vi "AR.Drone MAIN.vi"() -> ()   [LabVIEW 2014]
uses:
  Resources/Others/Control cluster.ctl
  <vilib>/LVH/AR Drone Toolkit/Decode NavData/Typedefs/NavData Demo.ctl
  Resources/Global.vi
  Kinect Extention/Kinect Global.vi
  <vilib>/LVH/AR Drone Toolkit/AR Drone.lvlib
panel:
  in  "Tab Control 3":enum32{"Flight Control"}(tab)
  in  "Manual":bool=TRUE
  in  "Switch control":bool
  in  "Enable Kinect Extention":bool
  in  "Tab Control 2":enum32{"Setup", "Debug&Test Info", "NavData"}(tab)
  in  "Enable Video":bool
  in  "Enable Controller Setup":bool
  in  "Reset OCR":bool
  in  "Secondary VI":u16(ring)=1 items=["Auto Hovering with Position Prediction.vi", "Simple Video.vi", "Circle detection.vi", "OCR Control.vi"]
  in  "Setup Parameters":T1={"Drone IP address"="192.168.1.1", "Home IP address"="192.168.1.2", "Flight Mode"=enum."INDOOR MODE", "Mounted Hull"=enum."INDOOR HULL", "Video Camera"=0, "Max Altitude (m)"=3.0, "Max Pitch and Roll Angle (deg)"=8.0, "Max Vertical Speed (m/s)"=0.7, "Max Yaw Speed (deg/s)"=100.0} {"Video Camera" items=["Bottom Camera"=1, "Front Camera"=0, "Front in Bottom"=3, "Bottom in Front"=2]}
  in  "Adjustments (affects Secondary VIs)":cluster{"Sensitivity":dbl, "Null Zone":dbl}={"Sensitivity"=1.0, "Null Zone"=1.0} {"Null Zone" scale=0.0..2.0; "Sensitivity" scale=0.0..2.0}
  in  "Enable Kinect Setup":bool
  out "Succesful Controller Setup":bool
  out "Succesful Drone Setup":bool
  in  "Control loop wait (ms)":u32=25
  out "Control loop Refesh Rate (ms)":u32
  in  "Video acquisition wait (ms)":u32=30
  out "Loop error":errorcluster
  out "Setup error":errorcluster
  out "Loop error (Ctr & Nav)":bool
  in  "Clear errors":bool
  out "Video procesing Refresh Rate (ms)":i32
  out "NavData Out":T2={"control state"=enum."INIT", "battery percentage"=100, "pitch (deg)"=0.0, "roll (deg)"=0.0, "yaw (deg)"=0.0, "altitude (cm)"=0, "vx (cm/s)?"=0.0, "vy (cm/s)?"=0.0, "vz (cm/s)?"=0.0, "detection cam type"=3}
  out "Battery Remaining":dbl(slide)=100.0 scale=0.0..100.0
  out "Hover (H)":bool
  out "Control Cluster":T3 {"Yaw Speed" scale=-1.0..1.0; "Vertical Speed" scale=-1.0..1.0; "Pitch" scale=-1.0..1.0; "Roll" scale=-1.0..1.0}
  out "Take off/Land (T)":bool
  in  "Tab Control":T4(tab)
  out "Raw":picture
  in  "Take photo":bool
  out "Generated path":path
  out "Error creating image":errorcluster
  out "Grayscale":T5(plugin-control)
  out "B&W":T5(plugin-control)
  in  "Calibrate Pitch":bool
  out "3D Picture":refnum<vi>(3d-picture)
  in  "stop":bool
  in  "Emergency Landing":bool
  # "Select Manual/Auto Control (based on Secondary VI)"
  # "Keyboard/Controller input"
  # "Enable Kinect gestuires (BETA)"
  # "(1 is default)"
  # "FOR ADVANCED USERS ONLY!"
  # "Not recommended!!!"
  # "This ignores the errors but does NOT eliminate them!"
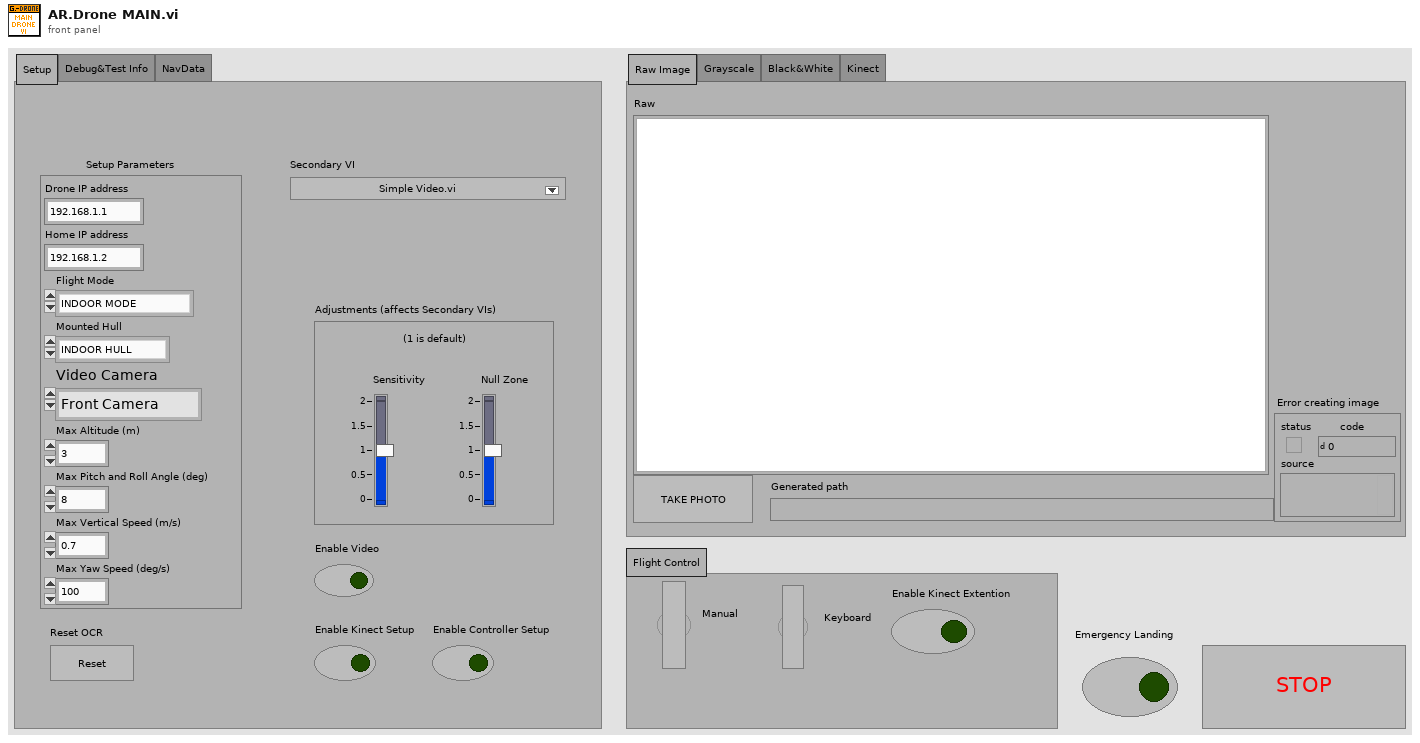
[diagram p1: front panel]
types:
  T1 = cluster{"Drone IP address":string, "Home IP address":string, "Flight Mode":enum8{"OUTDOOR MODE", "INDOOR MODE"}, "Mounted Hull":enum8{"OUTDOOR HULL", "INDOOR HULL"}, "Video Camera":u8, "Max Altitude (m)":sgl, "Max Pitch and Roll Angle (deg)":sgl, "Max Vertical Speed (m/s)":sgl, "Max Yaw Speed (deg/s)":sgl}
  T2 = typedef "AR Drone.lvlib/NavData Demo.ctl" = cluster{"control state":enum32{"DEFAULT", "INIT", "LANDING", "FLYING", "HOVERING", "TEST", "TRANS_TAKEOFF", "TRANS_GOTOFIX", "TRANS_LANDING"}, "battery percentage":u32, "pitch (deg)":sgl, "roll (deg)":sgl, "yaw (deg)":sgl, "altitude (cm)":u32, "vx (cm/s)?":sgl, "vy (cm/s)?":sgl, "vz (cm/s)?":sgl, "detection cam type":u32}
  T3 = typedef "Control cluster.ctl" = cluster{"Roll":sgl, "Pitch":sgl, "Vertical Speed":sgl, "Yaw Speed":sgl}
  T4 = enum32{"Raw Image", "Grayscale", "Black&White", "Kinect"}
  T5 = typedef "IMAQ Image.ctl" = refnum<image>
  T6 = typedef "imagedata.ctl" = cluster{"image type":i32, "image depth":i32, "image":u8[], "mask":u8[], "colors":u32[], "Rectangle":cluster{"left":i16, "top":i16, "right":i16, "bottom":i16}}
  T7 = typedef "AR Drone.lvlib/AR Drone Resource.ctl" = cluster{"UDP Control Connection":refnum<k16>, "UDP NavData Connection":refnum<k16>, "UDP Video Connection (Drone 1.0)":refnum<k16>, "TCP Video Connection (Drone 2.0)":refnum<k5>, "TCP Control Port Connection":refnum<k5>, "Drone IP address":string, "Drone Command Port":u16, "Drone NavData Port":u16, "Drone Vid Stream Port":u16, "Drone TCP Control Port":u16, "Home IP address":string, "Home Command Port":u16, "Home NavData Port":u16, "Home Vid Stream Port":u16, "Drone Version":i32, "Drone Index":i32, "Command Sequence":i32}
  T8 = cluster{"Roll":dbl, "Pitch":dbl, "Vertical Speed":dbl, "Yaw Speed":dbl}
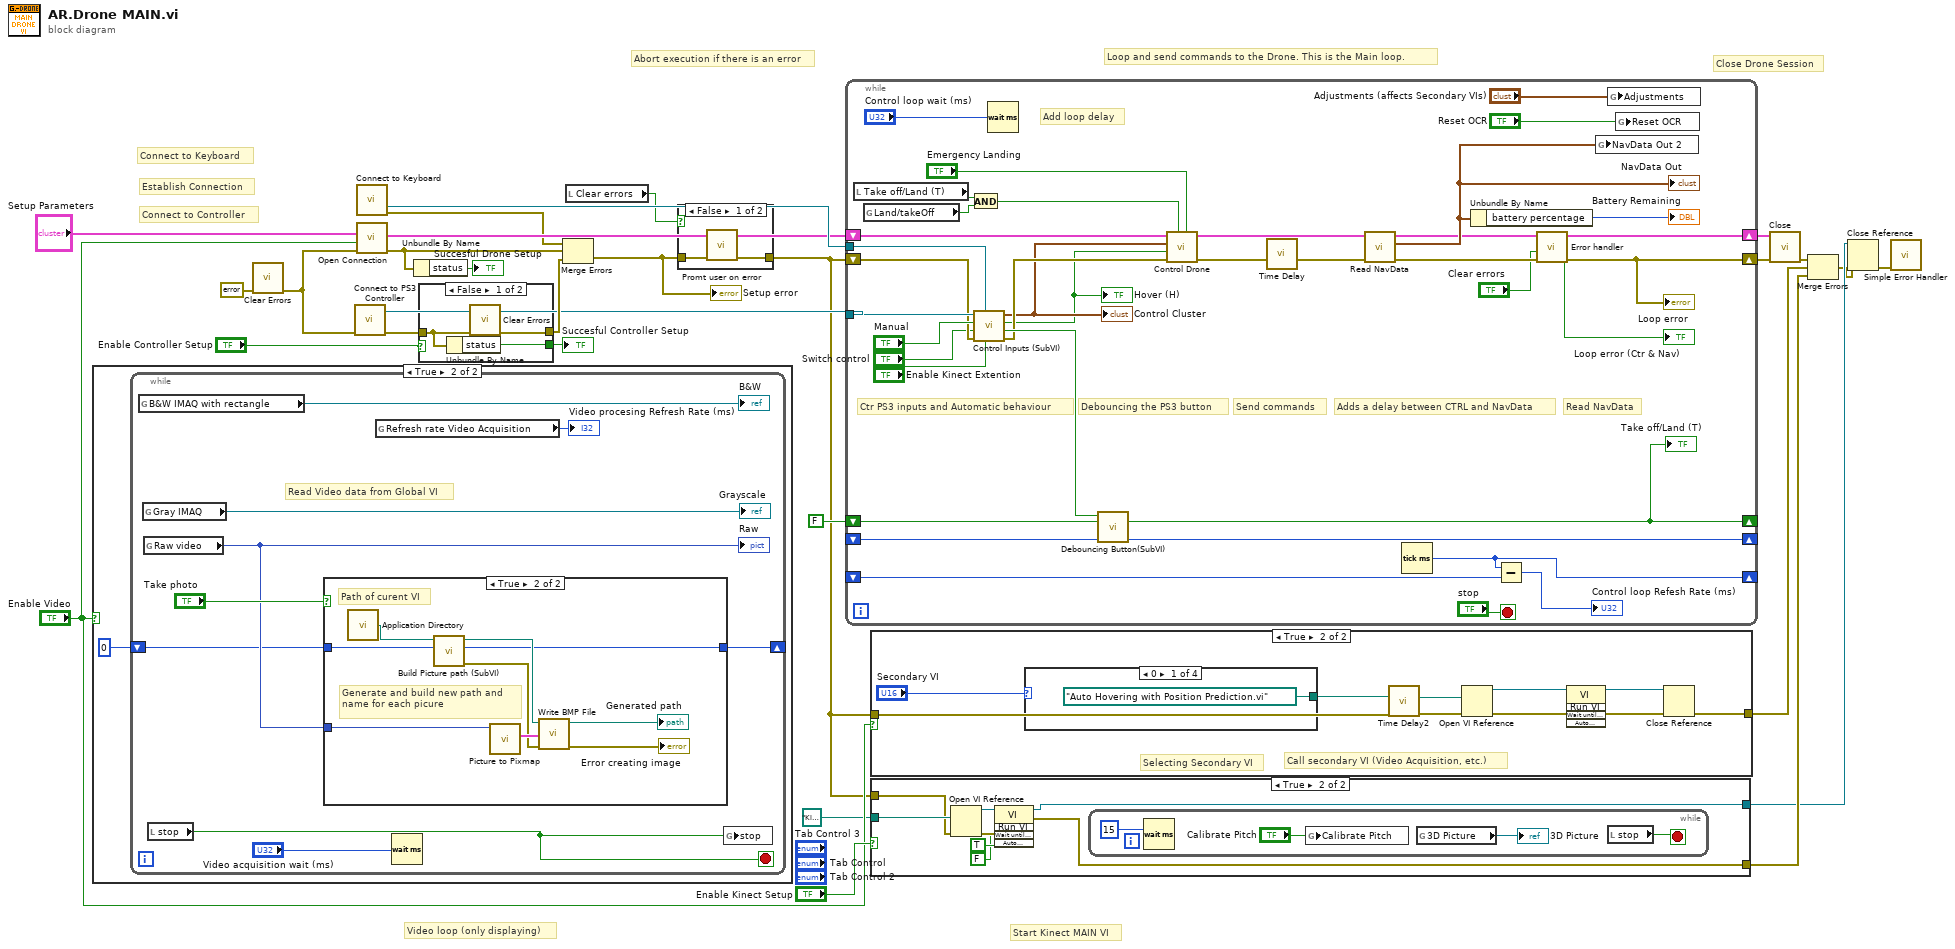
[diagram p0: block diagram]
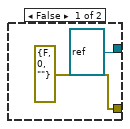
[diagram p2: hidden frame]
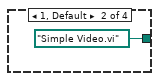
[diagram p4: hidden frame]
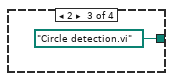
[diagram p5: hidden frame]
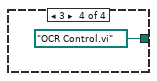
[diagram p6: hidden frame]
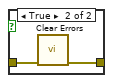
[diagram p9: hidden frame]
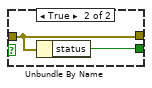
[diagram p10: hidden frame]
diagram:
  # "Start Kinect MAIN VI"
  # "Video loop (only displaying)"
  # "Connect to Keyboard"
  # "Connect to Controller"
  # "Abort execution if there is an error"
  # "Establish Connection"
  # "Close Drone Session"
  # "Loop and send commands to the Drone. This is the Main loop."
  n1 = case shown="True" "Enable Video" {
    frame False {
    }
    frame True {
      n2 = while {
        shift-right: [w31] -> _
        shift-left: 0 -> [w32]
        stop <- w38 stop-if-true
        # "Read Video data from Global VI"
        n3 = global read "Global.vi" "B&W IMAQ with rectangle"() -> (→"B&W":T5)
        n4 = global read "Global.vi" "Gray IMAQ"() -> (→"Grayscale":T5)
        n5 = global read "Global.vi" "Raw video"() -> (w33:picture)
        "Raw" <- w33
        n6 = local read "stop"() -> (w38:bool)
        n7 = case shown="True" "Take photo" {
          tunnel: w33 -> [_ w46]
          tunnel: w32 -> [w39 w44]
          tunnel: [w39 w43] -> w31
          frame False {
          }
          frame True {
            # "Generate and build new path and name for each picure"
            # "Path of curent VI"
            n8 = call <vilib>:"Application Directory.vi"() -> ("Application Directory"=w42:path)
            n9 = call "Build Picture path (SubVI).vi"("Numeric in"=w44, "Application Directory"=w42) -> ("Error Out"=w40:errorcluster, "Numeric out"=w43:i32, "Path"=w47:path)  [unwired: 7 in]
            n10 = call <vilib>:"Picture to Pixmap.vi"("picture"=w46) -> ("image data"=w48:T6)  [unwired: 9 in, 1 out]
            n11 = call <vilib>:"Write BMP File.vi"("error in (no error)"=w40, "image data"=w48, "path to BMP file"=w47) -> ("error out"=→"Error creating image":errorcluster, "path"=→"Generated path":path)  [unwired: 7 in]
          }
        }
        n12 = global read "Global.vi" "Refresh rate Video Acquisition"() -> (→"Video procesing Refresh Rate (ms)":i64)
        n13 = Wait (ms)(milliseconds to wait="Video acquisition wait (ms)") -> ()  [unwired: 1 out]
        n14 = global write "Global.vi" "stop"(w38) -> ()
      }
    }
  }
  n15 = call <vilib>:"Clear Errors.vi"("error in (no error)"=errorcluster {"status"=FALSE, "code"=0, "source"=""}) -> ("error out"=w16:errorcluster)  [unwired: 5 in, 1 out]
  n16 = call "Connect to PS3 Controller.vi"("error in (no error)"=w16) -> ("error out"=w14:errorcluster, "device ID 2"=w12:refnum<k1>)  [unwired: 8 in]
  n17 = call "Connect to Keyboard.vi"() -> ("device ID"=w20:refnum<k1>, "error out"=w17:errorcluster)  [unwired: 13 in, 1 out]
  n18 = call "Open Connection.vi"("error in (no error)"=w16, "Init Video?"="Enable Video", "Setup Parameters"="Setup Parameters") -> ("error out"=w18:errorcluster, "AR Drone Resource"=w19:T7)  [unwired: 7 in]
  n19 = Unbundle By Name(w18) -> ("status"=→"Succesful Drone Setup":bool)
  n20 = case shown="False" "Enable Controller Setup" {
    tunnel: w14 -> [w50 w53]
    tunnel: [w51 w53] -> w13
    tunnel: [w49 w52] -> w11
    frame False {
      n21 = Unbundle By Name(w50) -> ("status"=w49:bool)
      n22 = call <vilib>:"Clear Errors.vi"("error in (no error)"=w50) -> ("error out"=w51:errorcluster)  [unwired: 5 in, 1 out]
    }
    frame True {
      n23 = Unbundle By Name(w53) -> ("status"=w52:bool)
    }
  }
  "Succesful Controller Setup" <- w11
  n24 = Merge Errors(w17, w18, w13) -> (w9:errorcluster)
  "Setup error" <- w9
  n25 = local read "Clear errors"() -> (w10:bool)
  n26 = case shown="False" w10 {
    tunnel: w9 -> [w55 w57]
    tunnel: [w54 w56] -> w3
    frame False {
      n27 = call "Promt user on error.vi"("error in (no error)"=w55) -> ("error out"=w54:errorcluster)  [unwired: 10 in]
    }
    frame True {
      n28 = call <vilib>:"Clear Errors.vi"("error in (no error)"=w57) -> ("error out"=w56:errorcluster)  [unwired: 5 in, 1 out]
    }
  }
  n29 = while {
    shift-right: [w76] -> w28
    shift-left: w19 -> [w92]
    shift-right: [w60] -> w26
    shift-left: w3 -> [w72]
    shift-right: [w69] -> _
    shift-left: _ -> [w88]
    shift-right: [w85] -> _
    shift-left: FALSE -> [w86]
    shift-right: [w84] -> _
    shift-left: _ -> [w83]
    tunnel: w12 -> [w78]
    tunnel: w20 -> [w62]
    stop <- "stop" stop-if-true
    # "Add loop delay"
    # "Ctr PS3 inputs and Automatic behaviour"
    # "Read NavData"
    # "Send commands"
    # "Debouncing the PS3 button"
    # "Adds a delay between CTRL and NavData"
    n30 = local read "Take off/Land (T)"() -> (w67:bool)
    n31 = global read "Global.vi" "Land/takeOff"() -> (w68:bool)
    n32 = And(x=w67, y=w68) -> (x .and. y?=w79:bool)
    n33 = call "Control Inputs (SubVI).vi"("Enable Kinect Extention"="Enable Kinect Extention", "Keyboard ID"=w62, "error in (no error)"=w72, "Switch control"="Switch control", "Manual"="Manual", "Controller ID"=w78) -> ("error out"=w71:errorcluster, "Land/Take off"=w87:bool, "Hover Out"=w66:bool, "Control cluster"=w70:T8)  [unwired: 2 in]
    "Control Cluster" <- w70
    "Hover (H)" <- w66
    n34 = Wait (ms)(milliseconds to wait="Control loop wait (ms)") -> ()  [unwired: 1 out]
    n35 = call "Debouncing Button(SubVI).vi"("millisecond timer value in"=w83, "Boolean in"=w86, "Land/Take off"=w87) -> ("millisecond timer value out"=w84:u32, "Boolean out"=w85:bool)  [unwired: 7 in]
    "Take off/Land (T)" <- w85
    n36 = call <vilib>:"Control Drone.vi"("Emergency Landing"="Emergency Landing", "Takeoff/Land"=w79, "error in (no error)"=w71, "Hover"=w66, "Control Cluster"=w70, "AR Drone Resource"=w92) -> ("error out"=w74:errorcluster, "AR Drone Resource Out"=w91:T7)  [unwired: 4 in]
    n37 = call "Time Delay"("error in (no error)"=w74) -> ("error out"=w75:errorcluster)  [unwired: 10 in]
    n38 = call <vilib>:"Read NavData.vi"("error in (no error)"=w75, "AR Drone Resource"=w91) -> ("error out"=w61:errorcluster, "NavData Out"=w80:T2, "AR Drone Resource Out"=w76:T7)  [unwired: 7 in]
    "NavData Out" <- w80
    n39 = Tick Count (ms)() -> (millisecond timer value=w69:u32)
    n40 = Unbundle By Name(w80) -> ("battery percentage"=→"Battery Remaining":u32)
    n41 = Subtract(x=w69, y=w88) -> (x-y=→"Control loop Refesh Rate (ms)":u32)
    n42 = call "Error handler.vi"("error in (no error)"=w61, "Clear errors"="Clear errors") -> ("error out"=w60:errorcluster, "status"=→"Loop error (Ctr & Nav)":bool)  [unwired: 8 in]
    "Loop error" <- w60
    n43 = global write "Global.vi" "NavData Out 2"(w80) -> ()
    n44 = global write "Global.vi" "Adjustments"("Adjustments (affects Secondary VIs)") -> ()
    n45 = global write "Global.vi" "Reset OCR"("Reset OCR") -> ()
  }
  n46 = case shown="True" "Enable Video" {
    tunnel: [w94 w99] -> w23
    tunnel: w3 -> [w94 w95]
    frame False {
    }
    frame True {
      # "Selecting Secondary VI"
      # "Call secondary VI (Video Acquisition, etc.)"
      n47 = case shown="0" "Secondary VI" {
        tunnel: [path "Auto Hovering with Position Prediction.vi" ("Video Acquisition VI path") path "Simple Video.vi" ("Video Acquisition VI path") path "Circle detection.vi" ("Video Acquisition VI path") path "OCR Control.vi" ("Video Acquisition VI path")] -> w98
        frame 0 {
        }
        frame 1, Default {
        }
        frame 2 {
        }
        frame 3 {
        }
      }
      n48 = call "Time Delay2"("error in (no error)"=w95) -> ("error out"=w102:errorcluster)  [unwired: 10 in]
      n49 = Open VI Reference(vi path=w98, error in (no error)=w102) -> (vi reference=w97:refnum<vi>, error out=w96:errorcluster)  [unwired: 4 in]
      n50 = invoke class="VI" method="Run VI"(reference=w97, error in=w96) -> (reference out=w101:refnum<vi>, error out=w103:errorcluster)  [unwired: 3 in, 3 out]
      n51 = Close Reference(reference=w101, error in (no error)=w103) -> (error out=w99:errorcluster)
    }
  }
  n52 = case shown="True" "Enable Kinect Setup" {
    tunnel: [errorcluster {"status"=FALSE, "code"=0, "source"=""} ("error out") w115] -> w7
    tunnel: path "Kinect Extention/Kinect MAIN.vi" -> [_ w114]
    tunnel: [refnum<vi> refnum ("vi reference") w113] -> w4
    tunnel: w3 -> [_ w112]
    frame False {
    }
    frame True {
      n53 = Open VI Reference(vi path=w114, error in (no error)=w112) -> (vi reference=w117:refnum<vi>, error out=w116:errorcluster)  [unwired: 4 in]
      n54 = invoke on="Invoke Node" class="VI" method="Run VI"(reference=w117, error in=w116, "Wait until done"=FALSE ("Wait Until Done"), "Auto Dispose Ref"=TRUE ("Auto Dispose Reference")) -> (reference out=w113:refnum<vi>, error out=w115:errorcluster)  [unwired: 1 in, 3 out]
      n55 = while {
        stop <- w119 stop-if-true
        n56 = Wait (ms)(milliseconds to wait=u32 15) -> ()  [unwired: 1 out]
        n57 = global write "Kinect Global.vi" "Calibrate Pitch"("Calibrate Pitch") -> ()
        n58 = global read "Kinect Global.vi" "3D Picture"() -> (→"3D Picture":refnum<vi>)
        n59 = local read "stop"() -> (w119:bool)
      }
    }
  }
  n60 = call <vilib>:"Close.vi"("error in (no error)"=w26, "AR Drone Resource"=w28) -> ("error out"=w24:errorcluster)  [unwired: 9 in]
  n61 = Merge Errors(w24, w23, w7) -> (w2:errorcluster)
  n62 = Close Reference(reference=w4, error in (no error)=w2) -> (error out=w1:errorcluster)
  n63 = call <vilib>:"Simple Error Handler.vi"("error in (no error)"=w1) -> ()  [unwired: 4 in, 5 out]
